vi "to string.vi"(8 "error in":errorcluster, 11 "Submodule EOL configuration":refnum<class "Submodule EOL configuration.lvclass">) -> (0 "error out":errorcluster, 1 "data":string, 2 "version":string, 3 "Submodule EOL configuration out":refnum<class "Submodule EOL configuration.lvclass">)   [LabVIEW 2025, in "Submodule EOL.lvlib" / "Submodule EOL configuration.lvclass"]
doc: "Provides an interface for saving a module configuration to a file or other serialized data source. It is recommended that all children of this class store data in two sets--data required for its own initialization, and any data required for parent initialization--and that each implementation uses the <b>Call Parent Method</b> primitive to serialize parent information.Copyright 2017 National Instruments Corporation\n\nLicensed under the Apache License, Version 2.0 (the \"License\"); you may not use this file except in compliance with the License. You may obtain a copy of the License at http://www.apache.org/licenses/LICENSE-2.0\nUnless required by applicable law or agreed to in writing, software distributed under the License is distributed on an \"AS IS\" BASIS, WITHOUT WARRANTIES OR CONDITIONS OF ANY KIND, either express or implied. See the License for the specific language governing permissions and limitations under the License."
uses:
  Submodule EOL configuration.lvclass
  Submodule EOL configuration.lvclass/Submodule EOL configuration.ctl
  Users/Public/Documents/Sandia National Labs/TSS Plugin/CEF.lvlibp/serializable configuration/CEF_serializable configuration.lvclass
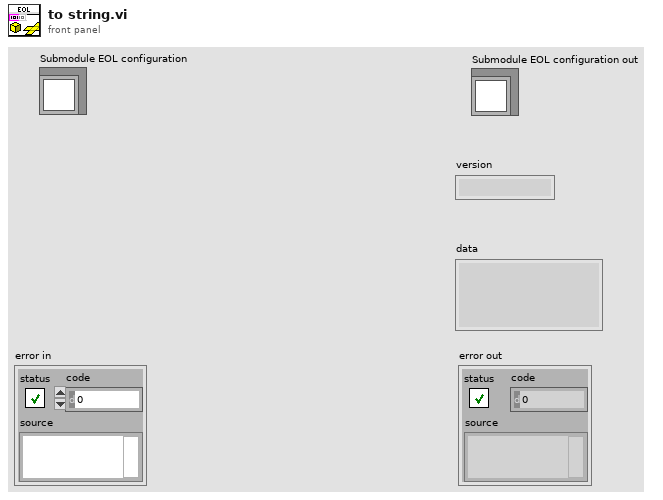
[diagram p1: front panel]
types:
  T1 = typedef "Submodule EOL.lvlib/Submodule EOL configuration.lvclass/Setting.ctl" = cluster{"Local Database":string, "Connect OPC Trial":u32, "Timeout Connect OPC":dbl, "AbstractUUT Path":string, "PreUUT Path":string, "Test Path":string, "PostUUT Path":string}
  T2 = typedef "Submodule EOL.lvlib/Submodule EOL configuration.lvclass/PLC.ctl" = cluster{"PLC Folder Names":string[][], "PLC URL":string, "Ignition Folder Names":string[][], "Ignition URL":string, "Test Name":string}
  T3 = typedef "Submodule EOL.lvlib/Submodule EOL configuration.lvclass/Instrumnet.ctl" = cluster{"Digitial IO":string, "HiPOT":string, "ACIR with Switch":string, "DMM with Switch":string}
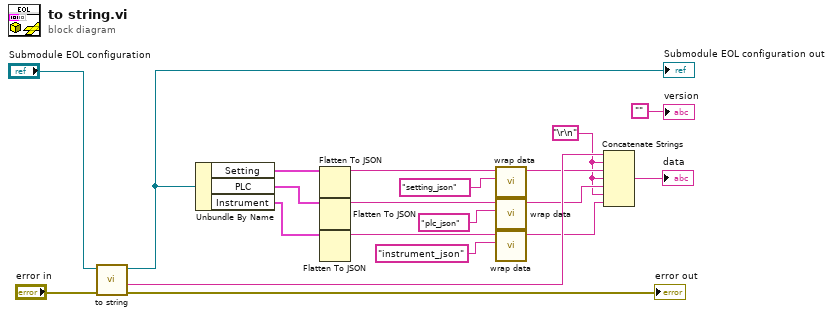
[diagram p0: block diagram]
diagram:
  w2 = "\r\n"
  n1 = call-parent "to string.vi"("error in"="error in", "CEF_Configuration"="Submodule EOL configuration") -> ("error out"=→"error out":errorcluster, "data"=w16:string, "CEF_Configuration out"=w13:refnum<class "Submodule EOL configuration.lvclass">)  [unwired: 6 in, 1 out]
  "Submodule EOL configuration out" <- w13
  n2 = Unbundle By Name(w13) -> ("Setting"=w19:T1, "PLC"=w10:T2, "Instrument"=w9:T3)
  n3 = Flatten To JSON(anything=w19) -> (JSON string=w17:string)  [unwired: 2 in, 1 out]
  n4 = Flatten To JSON(anything=w10) -> (JSON string=w8:string)  [unwired: 2 in, 1 out]
  n5 = Flatten To JSON(anything=w9) -> (JSON string=w6:string)  [unwired: 2 in, 1 out]
  n6 = call "wrap data.vi"("identifier"="setting_json" ("additional identifier"), "data to wrap"=w17) -> ("wrapped data"=w12:string)  [unwired: 9 in]
  n7 = call "wrap data.vi"("identifier"="plc_json" ("additional identifier"), "data to wrap"=w8) -> ("wrapped data"=w4:string)  [unwired: 9 in]
  n8 = call "wrap data.vi"("identifier"="instrument_json" ("additional identifier"), "data to wrap"=w6) -> ("wrapped data"=w3:string)  [unwired: 9 in]
  n9 = Concatenate Strings(w16, w2, w12, w2, w4, w2, w3) -> (→"data":string)
  "version" <- ""
